vi "Continuity_SMUResistanceTest.vi"(9 "DCPower_Parameters":T1={"Output"=enum."DC Voltage", "Current_range"=0.0, "Current"=0.0, "Voltage_range"=0.0, "Voltage"=0.0, "Aperture_time"=0.0, "Source Delay"=0.0, "Sense"=1008} {"Source Delay" format="%.6p"; "Sense" items=["Local"=1008, "Remote"=1009]; "Aperture_time" format="%.6p"; "Current_range" format="%.6p"; "Current" format="%.6p"; "Voltage_range" format="%.6p"; "Voltage" format="%.6p"}, 10 "Pins":T2[](array[typedef]), 11 "Semiconductor Module Context":T3) -> (0 "error out":errorcluster)   [LabVIEW 2023, in "Continuity.lvlib"]
doc: "Measures the resistance using an SMU channel in order to perform simple Continuity Test"
uses:
  Continuity.lvlib
  <vilib>/NI_TestStand_SemiconductorModule/NI_TestStand_Semiconductor_Module.lvlibp/PinMap/General/SemiconductorModuleContext.ctl
  <vilib>/NI_TestStand_SemiconductorModule/NI_TestStand_Semiconductor_Module.lvlibp/PinMap/TagProvider/TSM_Pin.ctl
  ResourceHandling/TypeDefs/RH_DCPower_Parameters.ctl
  <vilib>/NI_TestStand_SemiconductorModule/NI_TestStand_Semiconductor_Module.lvlibp/PinMap/PinQueryContext/MultiplePinMultipleSessionQueryContext/MultiplePinMultipleSessionQueryContext.lvclass
  C:/Program Files/National Instruments/LabVIEW 2023/vi.lib/NI_TestStand_SemiconductorModule/NI_TestStand_Semiconductor_Module.lvlibp/PinMap/PinQueryContext/PinQueryContext.lvclass
  <vilib>/NI_TestStand_SemiconductorModule/NI_TestStand_Semiconductor_Module.lvlibp/PinMap/DC Power/PinsToNIDCPowerSessions.vi
  <vilib>/NI_TestStand_SemiconductorModule/NI_TestStand_Semiconductor_Module.lvlibp/PinMap/General/Publish/PublishDataDouble1D.vi
  ResourceHandling/ResourceHandling.lvlib
  <vilib>/NI_TestStand_SemiconductorModule/NI_TestStand_Semiconductor_Module.lvlibp
  C:/Program Files/National Instruments/LabVIEW 2023/vi.lib/NI_TestStand_SemiconductorModule/NI_TestStand_Semiconductor_Module.lvlibp/PinMap/PinQueryContext/MultipleSessionPinQueryContext.lvclass
  C:/Program Files/National Instruments/LabVIEW 2023/vi.lib/NI_TestStand_SemiconductorModule/NI_TestStand_Semiconductor_Module.lvlibp/PinMap/PinQueryContext/MultiplePinMultipleSessionQueryContext/MultiplePinMultipleSessionQueryContext.lvclass
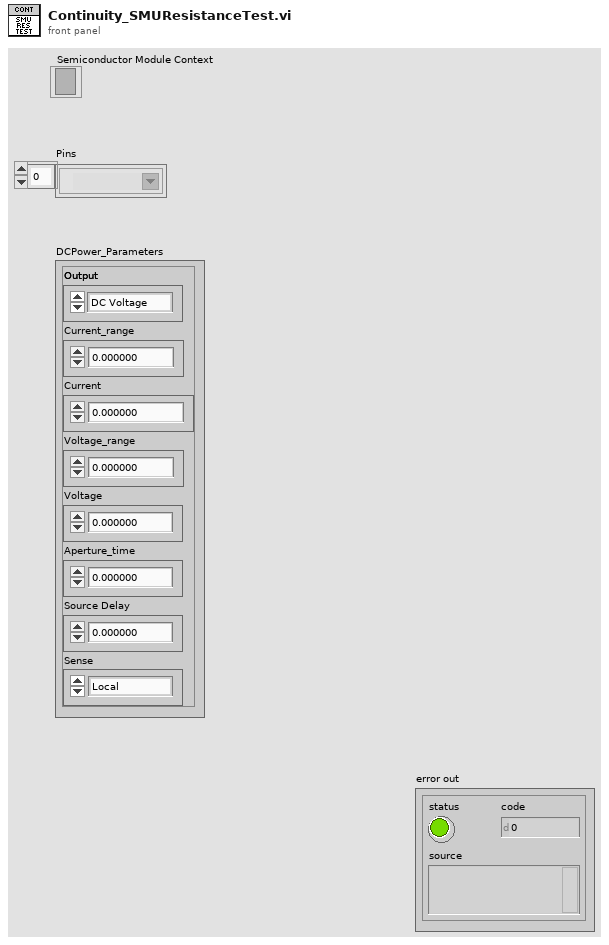
[diagram p1: front panel]
types:
  T1 = typedef "ResourceHandling.lvlib/RH_DCPower_Parameters.ctl" = cluster{"Output":enum16{"DC Voltage", "DC Current"}, "Current_range":dbl, "Current":dbl, "Voltage_range":dbl, "Voltage":dbl, "Aperture_time":dbl, "Source Delay":dbl, "Sense":i32}
  T2 = typedef "NI_TestStand_Semiconductor_Module.lvlibp/TSM_Pin.ctl" = tag
  T3 = typedef "NI_TestStand_Semiconductor_Module.lvlibp/SemiconductorModuleContext.ctl" = refnum<k7>
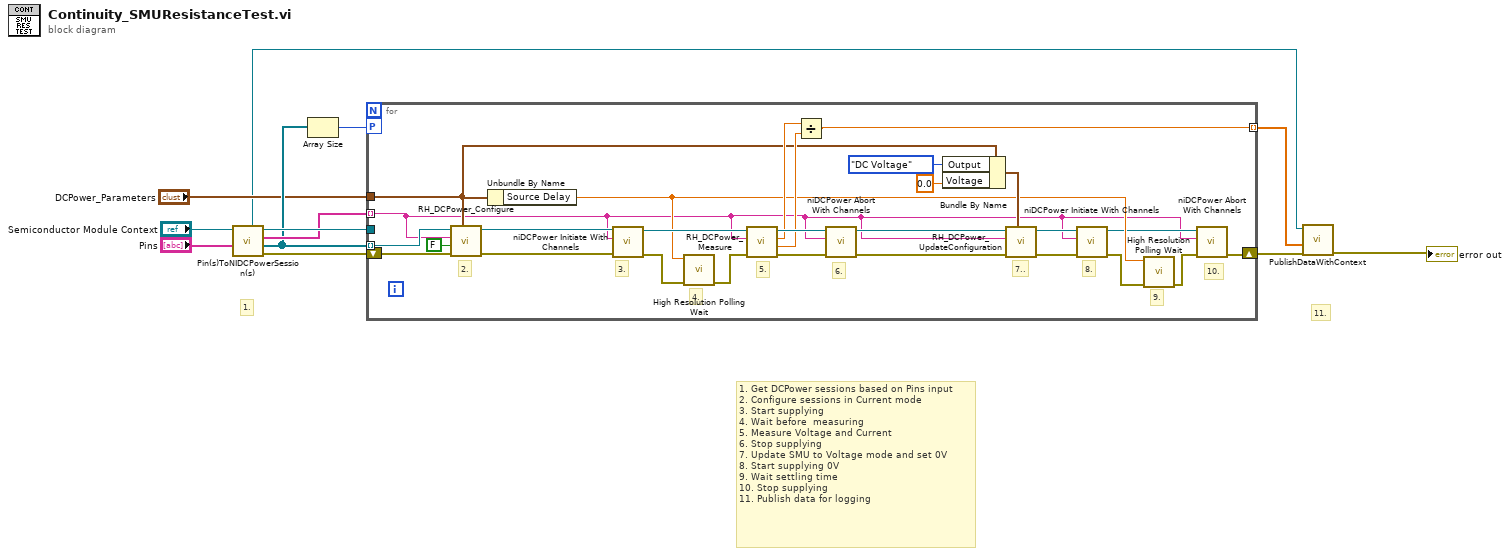
[diagram p0: block diagram]
diagram:
  # "11."
  # "1. Get DCPower sessions based on Pins input\n2. Configure sessions in Current mode\n3. Start supplying\n4. Wait before  measuring\n5. Measure Voltage and Current\n6. Stop supplying\n7. Update SMU to Voltage mode and set 0V\n8. Start supplying 0V\n9. Wait settling time\n10. Stop supplying\n11. Publish data for logging"
  # "1."
  n1 = call-poly <vilib>:"Pin(s)ToNIDCPowerSession(s).vi"("Pins"="Pins", "Semiconductor Module Context"="Semiconductor Module Context") -> ("error out"=w9:errorcluster, "Instrument Sessions"=w6:refnum<k15>[], "Channel Strings"=w8:string[], "Semiconductor Module Context Out"=w10:T3, "Pin Query Context"=w1:refnum<class "MultiplePinMultipleSessionQueryContext.lvclass">)  [unwired: 5 in]
  n2 = Array Size(array=w6) -> (size(s)=w7:i32)
  n3 = for {
    tunnel: w10 -> [_]
    shift-right: [w13] -> w4
    shift-left: w9 -> [w39]
    tunnel: w8 -> [w15] mode=indexing
    tunnel: w6 -> [w38] mode=indexing
    workers-P: w7 -> [_]
    tunnel: "DCPower_Parameters" -> [w25]
    tunnel: [w14] -> w2 mode=indexing
    # "10."
    # "9."
    # "8."
    # "7.."
    # "6."
    # "5."
    # "4."
    # "3."
    # "2."
    n4 = call "RH_DCPower_Configure.vi"("DCPower_Parameters"=w25, "error in (no error)"=w39, "trigger out?"=FALSE, "channel name"=w15, "DCPower Session In"=w38) -> ("error out"=w35:errorcluster, "DCPower Session Out"=w36:refnum<k15>)  [unwired: 5 in]
    n5 = Unbundle By Name(w25) -> ("Source Delay"=w18:dbl)
    n6 = call <instrlib>:"niDCPower Initiate With Channels.vi"("error in (no error)"=w35, "channel name"=w15, "instrument handle"=w36) -> ("error out"=w34:errorcluster, "instrument handle out"=w33:refnum<k15>)  [unwired: 7 in]
    n7 = call <vilib>:"High Resolution Polling Wait.vi"("error in (no error)"=w34, "seconds to wait"=w18) -> ("error out"=w32:errorcluster)  [unwired: 9 in]
    n8 = call "RH_DCPower_Measure.vi"("error in (no error)"=w32, "channel name"=w15, "DCPower Session In"=w33) -> ("error out"=w31:errorcluster, "Current"=w28:dbl, "Voltage"=w29:dbl, "DCPower Session Out"=w30:refnum<k15>)  [unwired: 5 in]
    n9 = Divide(x=w29, y=w28) -> (x/y=w14:dbl)
    n10 = call <instrlib>:"niDCPower Abort With Channels.vi"("error in (no error)"=w31, "channel name"=w15, "instrument handle"=w30) -> ("error out"=w27:errorcluster, "instrument handle out"=w26:refnum<k15>)  [unwired: 7 in]
    n11 = Bundle By Name(cluster=w25, "Output"=enum16{"DC Voltage", "DC Current"}."DC Voltage", "Voltage"=0.0) -> (w24:T1)
    n12 = call "RH_DCPower_UpdateConfiguration.vi"("DCPower_Parameters"=w24, "error in (no error)"=w27, "channel name"=w15, "DCPower Session In"=w26) -> ("error out"=w21:errorcluster, "DCPower Session Out"=w20:refnum<k15>)  [unwired: 6 in]
    n13 = call <instrlib>:"niDCPower Initiate With Channels.vi"("error in (no error)"=w21, "channel name"=w15, "instrument handle"=w20) -> ("error out"=w19:errorcluster, "instrument handle out"=w16:refnum<k15>)  [unwired: 7 in]
    n14 = call <vilib>:"High Resolution Polling Wait.vi"("error in (no error)"=w19, "seconds to wait"=w18) -> ("error out"=w17:errorcluster)  [unwired: 9 in]
    n15 = call <instrlib>:"niDCPower Abort With Channels.vi"("error in (no error)"=w17, "channel name"=w15, "instrument handle"=w16) -> ("error out"=w13:errorcluster)  [unwired: 7 in, 1 out]
  }
  n16 = call-poly <vilib>:"PublishDataWithContext.vi"("error in (no error)"=w4, "Data In"=w2, "Pin Query Context"=w1) -> ("error out"=→"error out":errorcluster)  [unwired: 7 in, 1 out]
